vi "VIH HelpGen - Build - Get Item Paths.vi"(8 "error in":errorcluster, 9 "Allowed files":path[](array[path]), 10 "Items Array":T4[](array[typedef]), 11 "Project Tree":T1) -> (0 "error out":errorcluster, 1 "Menus":T2, 2 "VIs":T3, 3 "dup Project Tree":T1, 4 "External":cluster{"Src Paths":path[], "Dst Paths":path[]})   [LabVIEW 2014]
doc: "::: VI Helpeks :::\nCopyright (c) 2000-2026 Konstantin Shifershteyn. All rights reserved."
uses:
  _VIH HelpGen - Palette.llb/VIH HelpGen Typedef - Palette - Item Info Cluster.ctl
  _VIH HelpGen - Palette.llb/VIH HelpGen Typedef - Palette - Item Type Enum.ctl
  _VIH Project Manager.llb/VIH Project Tree Typedef - Tree Refnum.ctl
  VIH HelpGen Typedef - Enum - Default,Enable,Disable.ctl
panel:
  # "VI Helpeks\nCopyright (c) 2012-2026 Konstantin Shifershteyn"
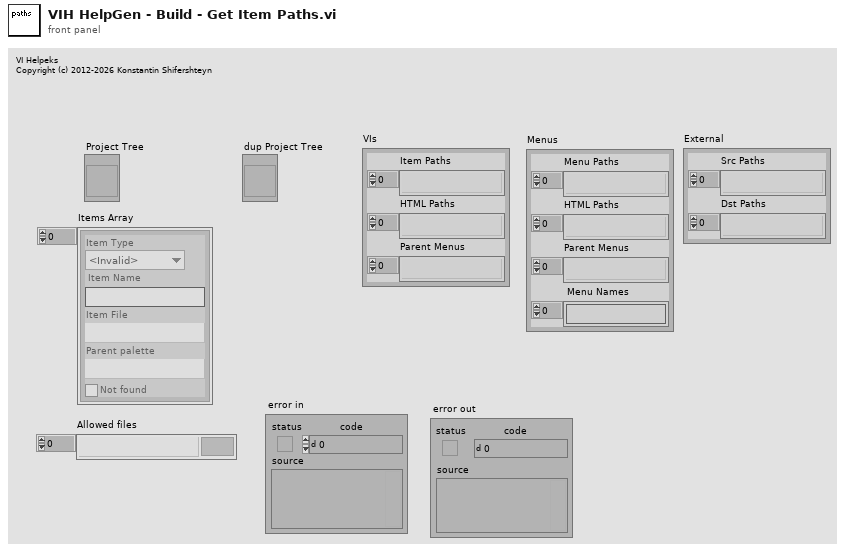
[diagram p1: front panel]
types:
  T1 = typedef "VIH Project Tree Typedef - Tree Refnum.ctl" = refnum<vi>
  T2 = cluster{"Menu Paths":path[], "HTML Paths":path[], "Parent Menus":path[], " Menu Names":string[]}
  T3 = cluster{"Item Paths":path[], "HTML Paths":path[], "Parent Menus":path[]}
  T4 = typedef "VIH HelpGen Typedef - Palette - Item Info Cluster.ctl" = cluster{"Item Type":T5, "Item Name":string, "Item File":path, "Parent palette":path, "Not found":bool}
  T5 = typedef "VIH HelpGen Typedef - Palette - Item Type Enum.ctl" = enum32{"<Invalid>", "<unknown>", "VI", "Menu", "LV Func", "Express VI", "Poly VI", "CTL", "HTML"}
  T6 = typedef "VIH HelpGen Typedef - Enum - Default,Enable,Disable.ctl" = enum16{"Default", "Enable", "Disable"}
  T7 = typedef "VIH HelpGen Typedef - Cluster - File Rule.ctl" = cluster{"OutName":string, "BuildHelp":T6, "Source Paths":T8, "Target Paths":T9, "DscrMode":T10, "Description":string, "Control Rules":T11[], "Flags":T13, "Ctl_DscrMode":T10, "Ctl_ClustMembers":T6, "Ctl_EnumValues":T6, "MenuItemIcons":T6, "%Comments":string, "DetailsMode":T10, "DetailsText":string, "ProductInfoMode":T6, "ProductInfoText":string}
  T8 = typedef "VIH HelpGen Typedef - Cluster - File Rule - Source Paths.ctl" = cluster{"CSS Files":path[], "JS Files":path[], "Html Template":path}
  T9 = typedef "VIH HelpGen Typedef - Cluster - File Rule - Target Paths.ctl" = cluster{"HTML Dir":path, "Image Dir":path, "CSS Dir":path, "JS Dir":path}
  T10 = typedef "VIH HelpGen Typedef - Enum - Description Mode.ctl" = enum16{"Default", "Description", "Description1", "Description2", "Custom", "None"}
  T11 = typedef "VIH HelpGen Typedef - Cluster - Control Rule.ctl" = cluster{"CtrlID":string, "CustomRule":bool, "DscrMode":T10, "Description":string, "ClusterMembers":T6, "EnumValues":T6, "EnumValDscr":T12[], "CustomName":string}
  T12 = typedef "VIH HelpGen Typedef - Cluster - Enum Value Info.ctl" = cluster{"Value":ext, "String":string, "Description":string}
  T13 = typedef "VIH HelpGen Typedef - Cluster - Group Rule - Flags.ctl" = cluster{"Override CSS Files":bool, "Override JS Files":bool, "Override Ctl Rules":bool}
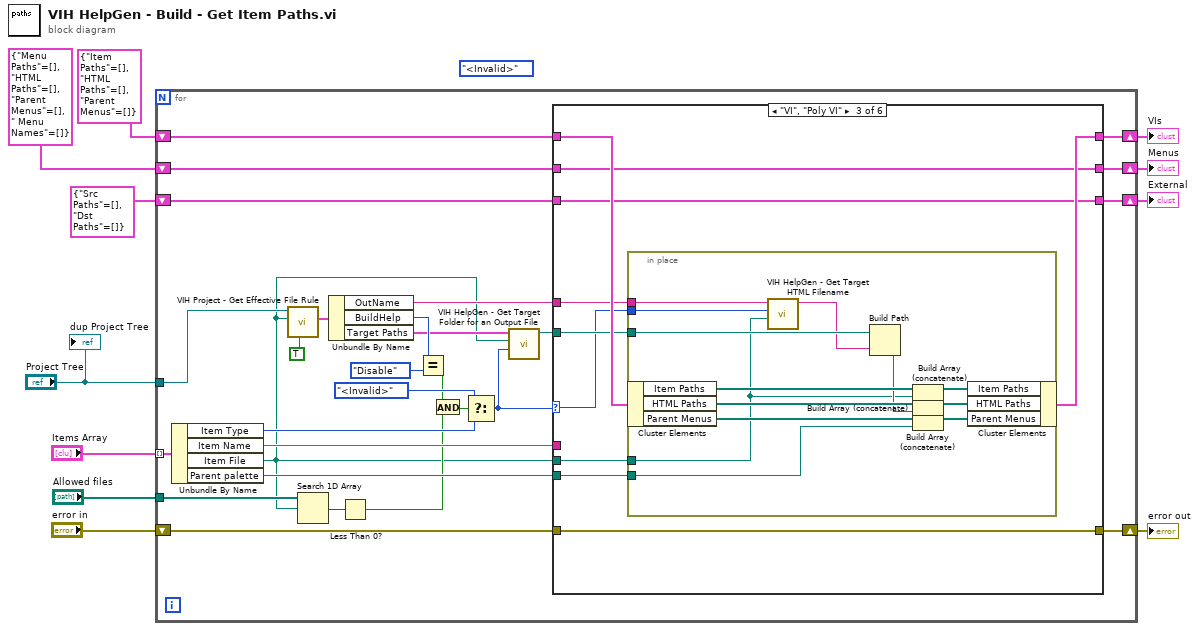
[diagram p0: block diagram]
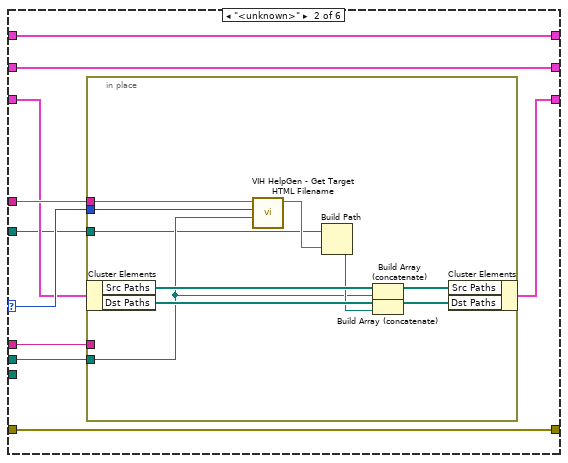
[diagram p3: hidden frame]
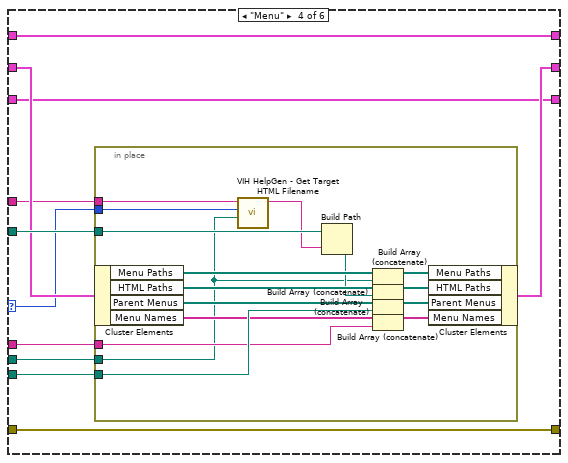
[diagram p4: hidden frame]
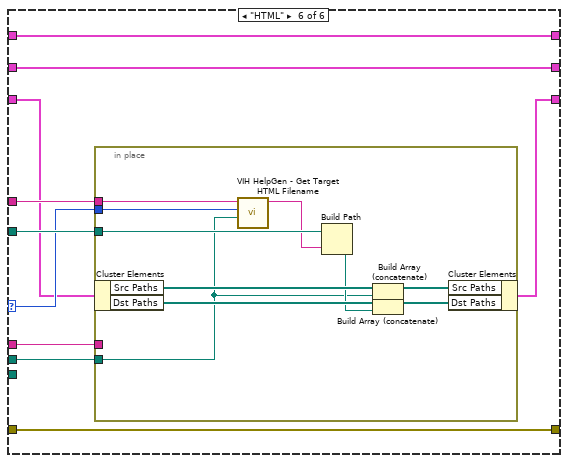
[diagram p6: hidden frame]
diagram:
  (unwired) VIH_HelpGen_Typedef_-_Palette_-_Item_Type_Enum."<Invalid>" ("t")
  n1 = for {
    tunnel: "Items Array" -> [w39] mode=indexing
    shift-right: [w37] -> w10
    shift-left: T3 {"Item Paths"=[], "HTML Paths"=[], "Parent Menus"=[]} ("VIs") -> [w38]
    shift-right: [w34] -> w7
    shift-left: T2 {"Menu Paths"=[], "HTML Paths"=[], "Parent Menus"=[], " Menu Names"=[]} ("Menus") -> [w35]
    shift-right: [w32] -> w5
    shift-left: "error in" -> [w33]
    tunnel: "Project Tree" -> [w30]
    tunnel: "Allowed files" -> [w24]
    shift-right: [w19] -> w2
    shift-left: cluster{"Src Paths":path[], "Dst Paths":path[]} {"Src Paths"=[], "Dst Paths"=[]} ("External") -> [w18]
    n2 = Unbundle By Name(w39) -> ("Item Type"=w27:T5, "Item Name"=w31:string, "Item File"=w13:path, "Parent palette"=w36:path)
    n3 = call "VIH Project - Get Effective File Rule.vi"("Ena <Invalid> (F)"=TRUE, "File Path"=w13, "Project Tree"=w30) -> ("Effective File Rule"=w17:T7)  [unwired: 5 in, 3 out]
    n4 = Search 1D Array(1D array=w24, element=w13) -> (index of element=w23:i32)  [unwired: 1 in]
    n5 = Unbundle By Name(w17) -> ("OutName"=w25:string, "BuildHelp"=w29:T6, "Target Paths"=w14:T9)
    n6 = Less Than 0?(x=w23) -> (x < 0?=w20:bool)
    n7 = Equal?(x=w29, y=VIH_HelpGen_Typedef_-_Enum_-_Default,Enable,Disable."Disable") -> (x = y?=w22:bool)
    n8 = And(x=w22, y=w20) -> (x .and. y?=w21:bool)
    n9 = Select(t=VIH_HelpGen_Typedef_-_Palette_-_Item_Type_Enum."<Invalid>", s=w21, f=w27) -> (s? t:f=w15:T5)
    n10 = call "VIH HelpGen - Get Target Folder for an Output File.vi"("Item/File Type"=w15, "File Path"=w13, "Target Paths"=w14) -> ("Target Folder"=w16:path)  [unwired: 8 in]
    n11 = case shown="\"VI\", \"Poly VI\"" w15 {
      selector: w15 -> [_ w48 w65 w88 _ w121]
      tunnel: w38 -> [w43 w52 w73 w94 w117 w125]
      tunnel: [w43 w52 w72 w94 w117 w125] -> w37
      tunnel: w13 -> [_ w53 w71 w97 _ w127]
      tunnel: w36 -> [_ _ w70 w96 _ _]
      tunnel: w16 -> [_ w44 w69 w95 _ w126]
      tunnel: w35 -> [w42 w47 w68 w93 w116 w120]
      tunnel: [w42 w47 w68 w92 w116 w120] -> w34
      tunnel: w33 -> [w41 w49 w67 w89 w115 w122]
      tunnel: [w41 w49 w67 w89 w115 w122] -> w32
      tunnel: w31 -> [_ w51 _ w91 _ w124]
      tunnel: w25 -> [_ w50 w66 w90 _ w123]
      tunnel: [w40 w45 w64 w87 w114 w118] -> w19
      tunnel: w18 -> [w40 w46 w64 w87 w114 w119]
      frame "<Invalid>", "LV Func" {
      }
      frame "<unknown>" {
        n12 = in-place {
          in-place-border: w53 -> [w55]
          in-place-border: w51 -> [_]
          in-place-border: w50 -> [w58]
          in-place-border: w48 -> [w56]
          in-place-border: w44 -> [w54]
          n13 = in-place-cluster #1(w46) -> ("Src Paths"=w63:path[], "Dst Paths"=w61:path[])
          n14 = call "VIH HelpGen - Get Target HTML Filename.vi"("Item File Path"=w55, "Item Type"=w56, "HTML Filename in"=w58) -> ("HTML Fileame out"=w57:string)  [unwired: 7 in, 1 out]
          n15 = Build Path(base path=w54, name or relative path=w57) -> (appended path=w59:path)
          n16 = Build Array (concatenate)(w63, w55) -> (w62:path[])
          n17 = Build Array (concatenate)(w61, w59) -> (w60:path[])
          n18 = in-place-cluster #1("Src Paths"=w62, "Dst Paths"=w60) -> (w45:cluster{"Src Paths":path[], "Dst Paths":path[]})
        }
      }
      frame "VI", "Poly VI" {
        n19 = in-place {
          in-place-border: w71 -> [w75]
          in-place-border: w70 -> [w80]
          in-place-border: w69 -> [w79]
          in-place-border: w66 -> [w77]
          in-place-border: w65 -> [w74]
          n20 = in-place-cluster #2(w73) -> ("Item Paths"=w86:path[], "HTML Paths"=w84:path[], "Parent Menus"=w83:path[])
          n21 = call "VIH HelpGen - Get Target HTML Filename.vi"("Item File Path"=w75, "Item Type"=w74, "HTML Filename in"=w77) -> ("HTML Fileame out"=w76:string)  [unwired: 7 in, 1 out]
          n22 = Build Path(base path=w79, name or relative path=w76) -> (appended path=w78:path)
          n23 = Build Array (concatenate)(w86, w75) -> (w85:path[])
          n24 = Build Array (concatenate)(w84, w78) -> (w82:path[])
          n25 = Build Array (concatenate)(w83, w80) -> (w81:path[])
          n26 = in-place-cluster #2("Item Paths"=w85, "HTML Paths"=w82, "Parent Menus"=w81) -> (w72:T3)
        }
      }
      frame "Menu" {
        n27 = in-place {
          in-place-border: w97 -> [w99]
          in-place-border: w96 -> [w107]
          in-place-border: w95 -> [w106]
          in-place-border: w91 -> [w102]
          in-place-border: w90 -> [w101]
          in-place-border: w88 -> [w98]
          n28 = in-place-cluster #3(w93) -> ("Menu Paths"=w113:path[], "HTML Paths"=w111:path[], "Parent Menus"=w110:path[], "Menu Names"=w104:string[])
          n29 = call "VIH HelpGen - Get Target HTML Filename.vi"("Item File Path"=w99, "Item Type"=w98, "HTML Filename in"=w101) -> ("HTML Fileame out"=w100:string)  [unwired: 7 in, 1 out]
          n30 = Build Path(base path=w106, name or relative path=w100) -> (appended path=w105:path)
          n31 = Build Array (concatenate)(w113, w99) -> (w112:path[])
          n32 = Build Array (concatenate)(w111, w105) -> (w109:path[])
          n33 = Build Array (concatenate)(w110, w107) -> (w108:path[])
          n34 = Build Array (concatenate)(w104, w102) -> (w103:string[])
          n35 = in-place-cluster #3("Menu Paths"=w112, "HTML Paths"=w109, "Parent Menus"=w108, "Menu Names"=w103) -> (w92:T2)
        }
      }
      frame "Express VI", "CTL" {
      }
      frame "HTML" {
        n36 = in-place {
          in-place-border: w127 -> [w129]
          in-place-border: w126 -> [w133]
          in-place-border: w124 -> [_]
          in-place-border: w123 -> [w131]
          in-place-border: w121 -> [w128]
          n37 = in-place-cluster #4(w119) -> ("Src Paths"=w137:path[], "Dst Paths"=w135:path[])
          n38 = call "VIH HelpGen - Get Target HTML Filename.vi"("Item File Path"=w129, "Item Type"=w128, "HTML Filename in"=w131) -> ("HTML Fileame out"=w130:string)  [unwired: 7 in, 1 out]
          n39 = Build Path(base path=w133, name or relative path=w130) -> (appended path=w132:path)
          n40 = Build Array (concatenate)(w137, w129) -> (w136:path[])
          n41 = Build Array (concatenate)(w135, w132) -> (w134:path[])
          n42 = in-place-cluster #4("Src Paths"=w136, "Dst Paths"=w134) -> (w118:cluster{"Src Paths":path[], "Dst Paths":path[]})
        }
      }
    }
  }
  "VIs" <- w10
  "Menus" <- w7
  "error out" <- w5
  "External" <- w2
  "dup Project Tree" <- "Project Tree"
